vi "set Marker Table OnOff.vi"(8 "error in (no error)":errorcluster, 10 "Marker Table On?":bool, 11 "Keysight 9020A in":refnum<class "Keysight 9020A.lvclass">) -> (0 "error out":errorcluster, 3 "Keysight 9020A out":refnum<class "Keysight 9020A.lvclass">)   [LabVIEW 2023, in "Spectrum Analyzer.lvlib" / "Keysight 9020A.lvclass"]
uses:
  Keysight 9020A.lvclass
  Keysight 9020A.lvclass/Keysight 9020A.ctl
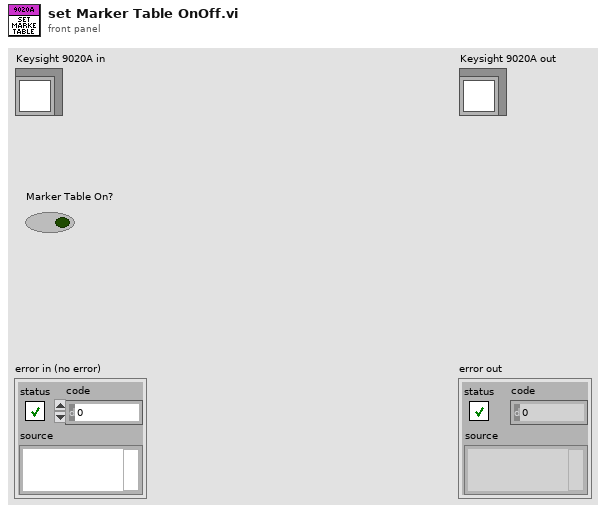
[diagram p1: front panel]
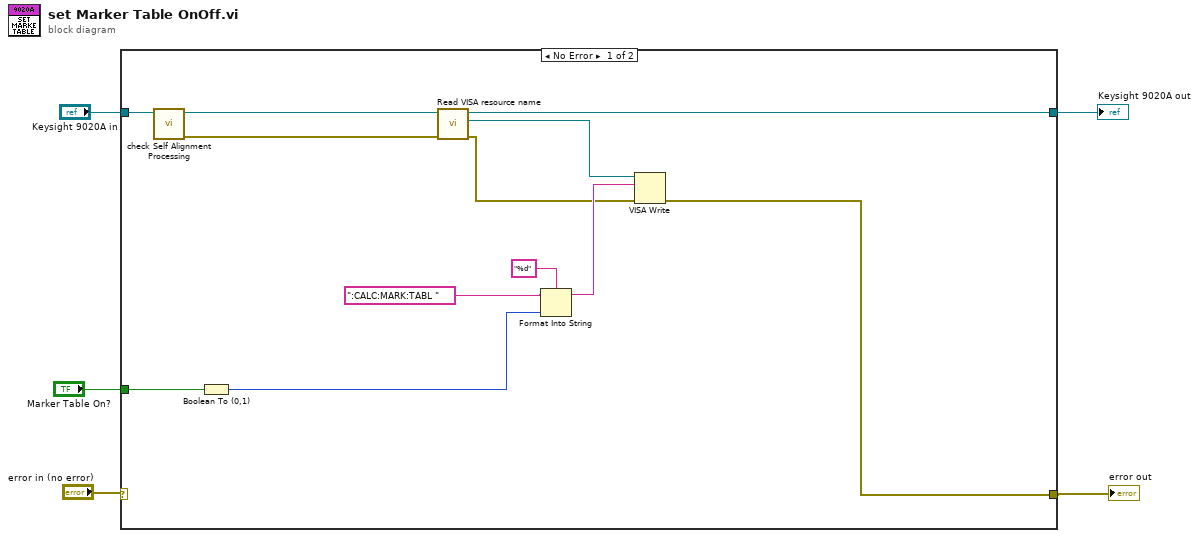
[diagram p0: block diagram]
diagram:
  n1 = case shown="No Error" "error in (no error)" {
    selector: "error in (no error)" -> [_ w18]
    tunnel: "Keysight 9020A in" -> [w12 w19]
    tunnel: [w13 w19] -> w4
    tunnel: [w15 w18] -> w2
    tunnel: "Marker Table On?" -> [w7 _]
    frame No Error {
      n2 = call "check Self Alignment Processing.vi"("Keysight 9020A in"=w12) -> ("error out"=w10:errorcluster, "Keysight 9020A out"=w11:refnum<class "Keysight 9020A.lvclass">)  [unwired: 8 in, 1 out]
      n3 = Boolean To (0,1)(Boolean=w7) -> (0, 1=w6:i16)
      n4 = call "Read VISA resource name.vi"("error in (no error)"=w10, "Keysight 9020A in"=w11) -> ("error out"=w9:errorcluster, "VISA resource name"=w14:refnum<visa-resource-name>, "Keysight 9020A out"=w13:refnum<class "Keysight 9020A.lvclass">)  [unwired: 7 in]
      n5 = Format Into String(format string="%d", initial string=":CALC:MARK:TABL ", w6) -> (resulting string=w17:string)  [unwired: 1 in, 1 out]
      n6 = VISA Write(VISA resource name=w14, write buffer=w17, error in (no error)=w9) -> (error out=w15:errorcluster)  [unwired: 2 out]
    }
    frame Error {
    }
  }
  "error out" <- w2
  "Keysight 9020A out" <- w4
